vi "GenNewTraj.vi"(6 "Drive Type":T1, 8 "Stoopid Overlap %":dbl min=0.0, 9 "Path Type":T6, 10 "Parameters":T5 {"Limits"."StoopidFast (fps)" min=0.0; "Limits"."Jerk (fps^3)" min=0.0 step=1.0; "Limits"."Accel (fps^2)" min=0.0; "Limits"."Velocity (fps)" min=0.0; "Overrides"."Angle Override" step=5.0; "Overrides"."Velocity Override" step=5.0; "Overrides"."Angular Override" step=5.0; "Angular Limits"."Jerk (deg/s^3)" min=0.0 step=1.0; "Angular Limits"."Accel (deg/s^2)" min=0.0; "Angular Limits"."Velocity (deg/s)" min=0.0}, 11 "Points in":cluster{"x":dbl, "y":dbl, "th":dbl}[](array[cluster])) -> (0 "Time & Dist":cluster{"Time (s)":dbl, "Distance (ft)":dbl}, 1 "Valid":bool, 2 "Trajectory Data":T7, 3 "Updated Waypoints":cluster{"x":dbl, "y":dbl, "th":dbl}[](array[cluster]))   [LabVIEW 2023]
uses:
  Types/Trajectory Data.ctl
  Types/Segment Type.ctl
  Types/Path Type.ctl
  Types/Limits.ctl
  Types/Overrides.ctl
  Types/Angluar Limits.ctl
  Types/Drive Type.ctl
  Bezier/Bezier Trajectory.vi
  Clothoid/Generate Clothoid Trajectory.vi
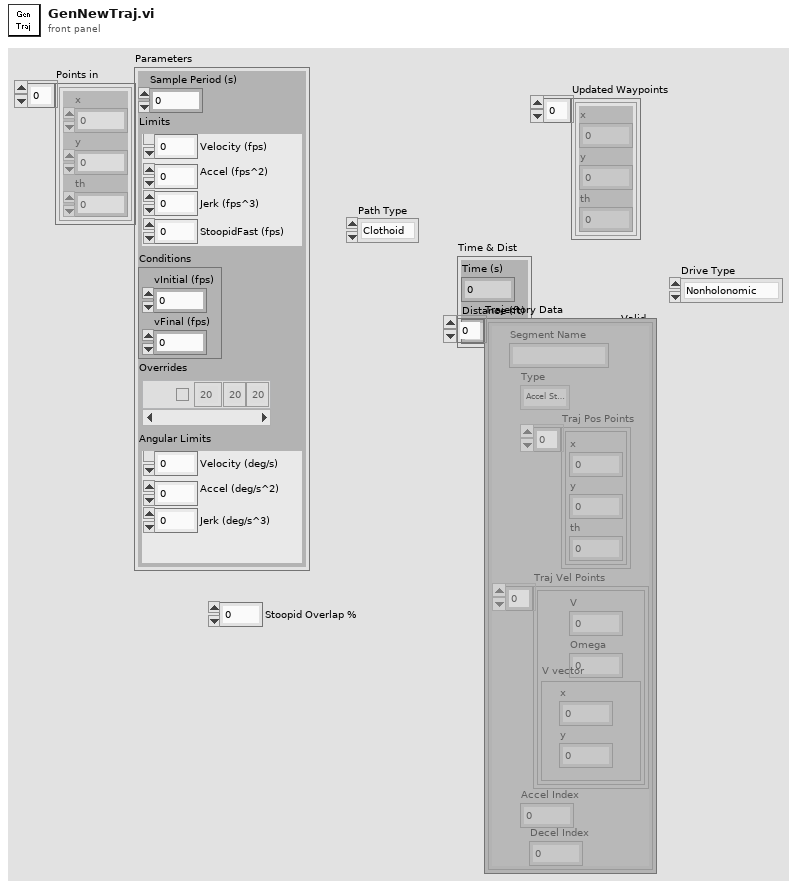
[diagram p1: front panel]
types:
  T1 = typedef "Drive Type.ctl" = enum16{"Nonholonomic", "Holonomic"}
  T2 = typedef "Limits.ctl" = cluster{"Velocity (fps)":dbl, "Accel (fps^2)":dbl, "Jerk (fps^3)":dbl, "StoopidFast (fps)":dbl}
  T3 = typedef "Overrides.ctl" = cluster{"Count":string, "Angular Override":dbl, "Enabled?":bool, "Velocity Override":dbl, "Angle Override":dbl}[]
  T4 = typedef "Angluar Limits.ctl" = cluster{"Velocity (deg/s)":dbl, "Accel (deg/s^2)":dbl, "Jerk (deg/s^3)":dbl}
  T5 = cluster{"Sample Period (s)":dbl, "Limits":T2, "Conditions":cluster{"vInitial (fps)":dbl, "vFinal (fps)":dbl}, "Overrides":T3, "Angular Limits":T4}
  T6 = typedef "Path Type.ctl" = enum16{"Clothoid", "Bezier"}
  T7 = typedef "Trajectory Data.ctl" = cluster{"Segment Name":string, "Type":T8, "Traj Pos Points":cluster{"x":dbl, "y":dbl, "th":dbl}[], "Traj Vel Points":cluster{"V":dbl, "Omega":dbl, "V vector":cluster{"y":dbl, "x":dbl}}[], "Accel Index":i32, "Decel Index":i32}[]
  T8 = typedef "Segment Type.ctl" = enum16{"Accel Straight", "Const Straight", "Blend", "Circle", "Bezier"}
  T9 = cluster{"vInitial (fps)":dbl, "vFinal (fps)":dbl}
  T10 = cluster{"Segment Name":string, "Type":T8, "Traj Pos Points":cluster{"x":dbl, "y":dbl, "th":dbl}[], "Traj Vel Points":cluster{"V":dbl, "Omega":dbl, "V vector":cluster{"y":dbl, "x":dbl}}[], "Accel Index":i32, "Decel Index":i32}[]
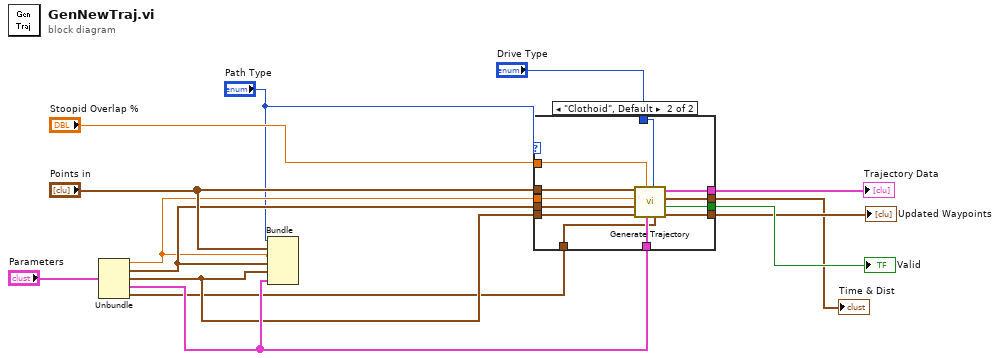
[diagram p0: block diagram]
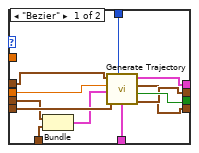
[diagram p2: hidden frame]
diagram:
  n1 = Unbundle("Parameters") -> ("Sample Period (s)"=w6:dbl, "Limits"=w9:T2, "Conditions"=w8:T9, "Overrides"=w11:T3, "Angular Limits"=w2:T4)
  n2 = Bundle("Path Type"="Path Type", "Points in"="Points in", "Sample Period (s)"=w6, "Limits"=w9, "Conditions"=w8, "Overrides"=w11) -> ()  [unwired: 1 in, 1 out]
  n3 = case shown="\"Clothoid\", Default" "Path Type" {
    tunnel: [w23 w38] -> w14
    tunnel: [w21 w37] -> w7
    tunnel: w8 -> [w25 w36]
    tunnel: w9 -> [w17 w35]
    tunnel: w11 -> [w24 w34]
    tunnel: [w20 w33] -> w13
    tunnel: [w22 w28] -> w5
    tunnel: "Stoopid Overlap %" -> [_ w32]
    tunnel: "Points in" -> [w26 w31]
    tunnel: w6 -> [w19 w30]
    tunnel: "Drive Type" -> [w18 w29]
    tunnel: w2 -> [w16 w27]
    frame "Bezier" {
      n4 = Bundle("Limits"=w17, "Angular Limits"=w16) -> (w15:cluster{"Limits":T2, "Angular Limits":T4})  [unwired: 1 in]
      n5 = call-poly "Generate Trajectory.vi"("Overrides"=w24, "Drive Type"=w18, "Conditions"=w25, "All Limits"=w15, "sample period (s)"=w19, "WayPoints"=w26) -> ("Time & Dist"=w21:cluster{"Time (s)":dbl, "Distance (ft)":dbl}, "Valid"=w23:bool, "Updated Waypoints"=w20:cluster{"x":dbl, "y":dbl, "th":dbl}[], "Trajectory Data"=w22:T7)  [unwired: 2 in]
    }
    frame "Clothoid", Default {
      n6 = call-poly "Generate Trajectory.vi"("Angular Limits"=w27, "Drive Type"=w29, "Overrides"=w34, "Stoopid Overlap %"=w32, "Conditions"=w36, "Limits"=w35, "Sample Period (s)"=w30, "WayPoints"=w31) -> ("Updated Waypoints"=w33:cluster{"x":dbl, "y":dbl, "th":dbl}[], "Valid"=w38:bool, "Time & Dist"=w37:cluster{"Time (s)":dbl, "Distance (ft)":dbl}, "Trajectory Data Out"=w28:T10)
    }
  }
  "Valid" <- w14
  "Updated Waypoints" <- w13
  "Time & Dist" <- w7
  "Trajectory Data" <- w5
